vi "SensorLogicSequence.vi"(1 "Turn Power":dbl=30.0, 2 "Port 2":T3 items=["Port 1", "Port 2", "Port 3", "Port 4"], 3 "Port 1":T3 items=["Port 1", "Port 2", "Port 3", "Port 4"], 4 "Movement Power":dbl=30.0, 5 "NXT/EV3 IN":T2, 7 "Black Threshold":sgl=20.0, 8 "Motor IDs":cluster{"Motors":T1, "Motors 2":T1}={"Motors"=0, "Motors 2"=1} {"Motors 2" items=["Port A", "Port B", "Port C", "Port D"]; "Motors" items=["Port A", "Port B", "Port C", "Port D"]}) -> (0 "NXT/EV3 OUT":T2)   [LabVIEW 2016, in "13.03 Robot.lvrbt"]
uses:
  13.03 Robot.lvrbt
  <vilib>/NXT/Block Support/NXT_InputPort.ctl
  <vilib>/NXT/Subs/LVHSConnector.ctl
  <vilib>/NXT/LegoClasses/BrickReference/BrickReference.lvclass
  <vilib>/NXT/Block Support/NXT_OutputPort.ctl
  <vilib>/NXT/Dual Mode Library/Display/drawText.vi
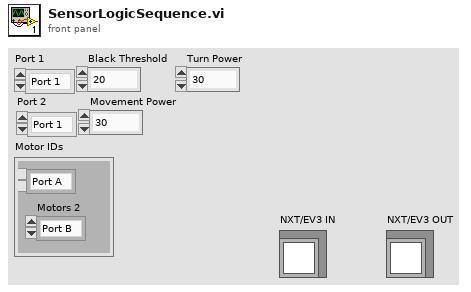
[diagram p1: front panel]
types:
  T1 = typedef "NXT_OutputPort.ctl" = u8
  T2 = typedef "LVHSConnector.ctl" = refnum<class "BrickReference.lvclass">
  T3 = typedef "NXT_InputPort.ctl" = u32
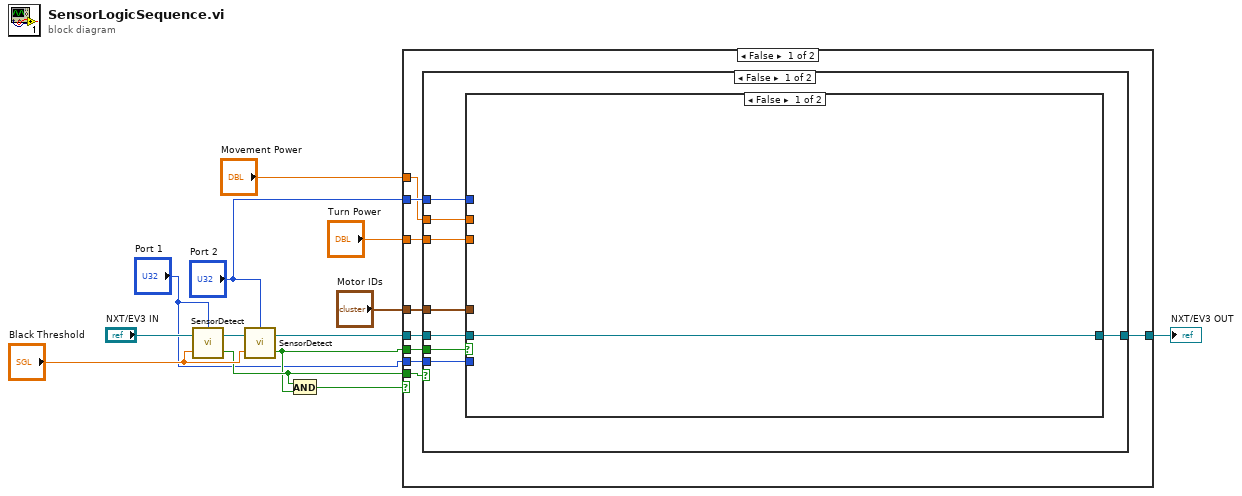
[diagram p0: block diagram]
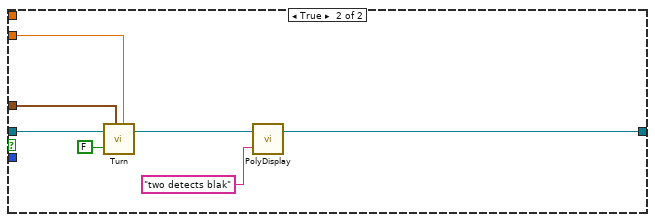
[diagram p2: hidden frame]
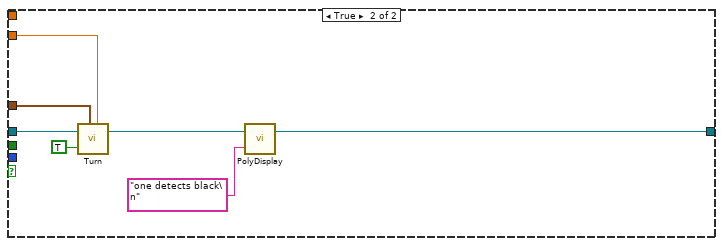
[diagram p3: hidden frame]
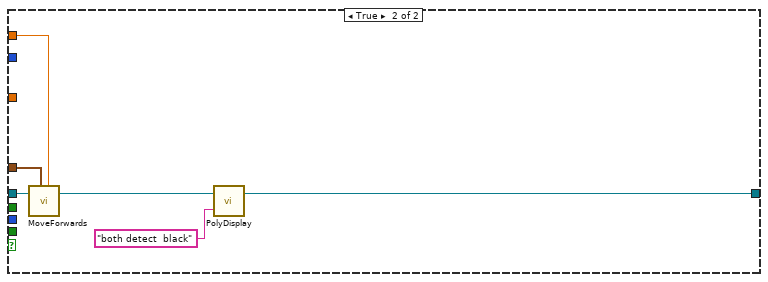
[diagram p4: hidden frame]
diagram:
  n1 = call "SensorDetect.vi"("Threshold"="Black Threshold", "NXT/EV3 IN"="NXT/EV3 IN", "Port (Port 1)"="Port 1") -> ("Out"=w5:bool, "NXT/EV3 OUT"=w13:T2)
  n2 = call "SensorDetect.vi"("Threshold"="Black Threshold", "NXT/EV3 IN"=w13, "Port (Port 1)"="Port 2") -> ("Out"=w3:bool, "NXT/EV3 OUT"=w8:T2)
  n3 = And(x=w5, y=w3) -> (x .and. y?=w10:bool)
  n4 = case shown="False" w10 {
    tunnel: "Movement Power" -> [w14 w51]
    tunnel: w8 -> [w21 w50]
    tunnel: "Motor IDs" -> [w20 w49]
    tunnel: [w18 w46] -> w6
    tunnel: w5 -> [w22 _]
    tunnel: "Turn Power" -> [w19 _]
    tunnel: w3 -> [w17 _]
    tunnel: "Port 1" -> [w16 _]
    tunnel: "Port 2" -> [w15 _]
    frame False {
      n5 = case shown="False" w22 {
        tunnel: w21 -> [w27 w44]
        tunnel: w20 -> [w29 w43]
        tunnel: w19 -> [w28 w42]
        tunnel: [w26 w39] -> w18
        tunnel: w17 -> [w30 _]
        tunnel: w16 -> [w25 _]
        tunnel: w15 -> [w24 _]
        tunnel: w14 -> [w23 _]
        frame False {
          n6 = case shown="False" w30 {
            tunnel: w29 -> [_ w38]
            tunnel: w28 -> [_ w37]
            tunnel: w27 -> [w31 w36]
            tunnel: [w31 w32] -> w26
            tunnel: w25 -> [_ _]
            tunnel: w24 -> [_ _]
            tunnel: w23 -> [_ _]
            frame False {
            }
            frame True {
              n7 = call "Turn.vi"("T - 1st, F - 2nd"=FALSE, "NXT/EV3 IN"=w36, "Motor IDs"=w38, "Power"=w37) -> ("NXT/EV3 OUT"=w33:T2)
              n8 = call-poly <vilib>:"PolyDisplay.vi"("Text"="two detects blak", "NXT/EV3"=w33) -> ("NXT/EV3"=w32:T2)  [unwired: 2 in]
            }
          }
        }
        frame True {
          n9 = call "Turn.vi"("T - 1st, F - 2nd"=TRUE, "NXT/EV3 IN"=w44, "Motor IDs"=w43, "Power"=w42) -> ("NXT/EV3 OUT"=w41:T2)
          n10 = call-poly <vilib>:"PolyDisplay.vi"("Text"="one detects black\n", "NXT/EV3"=w41) -> ("NXT/EV3"=w39:T2)  [unwired: 2 in]
        }
      }
    }
    frame True {
      n11 = call "MoveForwards.vi"("NXT/EV3 IN"=w50, "Motor IDs"=w49, "Power"=w51) -> ("NXT/EV3 OUT"=w47:T2)  [unwired: 1 in]
      n12 = call-poly <vilib>:"PolyDisplay.vi"("Text"="both detect  black", "NXT/EV3"=w47) -> ("NXT/EV3"=w46:T2)  [unwired: 2 in]
    }
  }
  "NXT/EV3 OUT" <- w6
